vi "Set Data Channel Property - ALL.vi"(8 "error in":errorcluster, 10 "Item Informations array":T2[](array[typedef]), 11 "Item Ref in":T1 format="%.0x") -> (0 "error out":errorcluster)   [LabVIEW 2023, in "Vires VTD System Explorer.lvlib"]
uses:
  Vires VTD System Explorer.lvlib
  Item Informations.ctl
  <vilib>/NI VeriStand/Custom Device API/Custom Device Item Info.ctl
  <vilib>/NI VeriStand/Custom Device API/Custom Device Channel.ctl
  <vilib>/NI VeriStand/Custom Device API/Custom Device Channel Type.ctl
  Data Channel Custom Property.ctl
  <vilib>/NI VeriStand/Custom Device API/Custom Device Item Ref.ctl
  Shared/Constants.vi
  <vilib>/NI VeriStand/Custom Device API/Custom Device API.lvlib
  Shared/Vires VTD Shared.lvlib
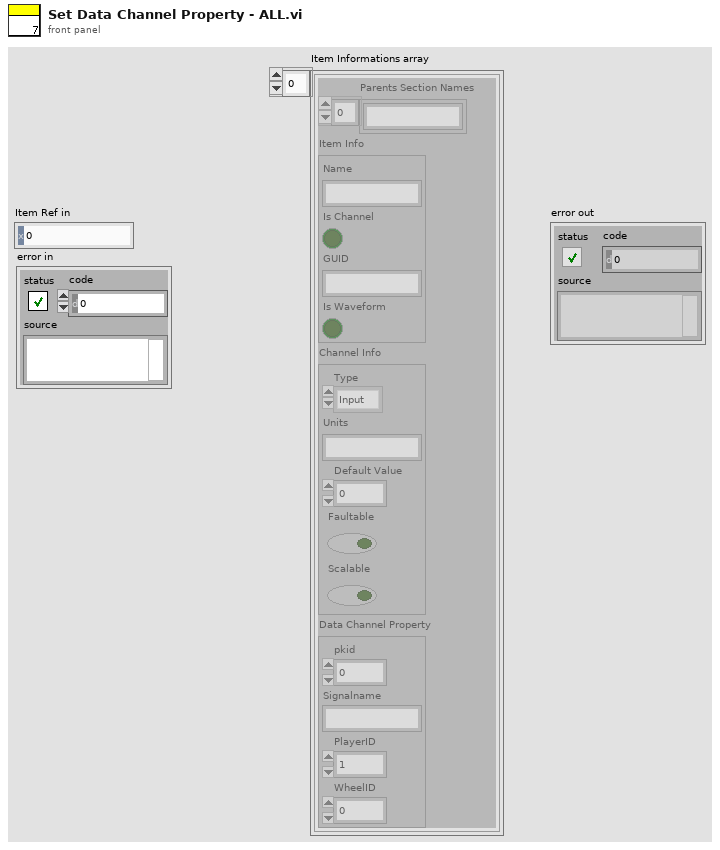
[diagram p1: front panel]
types:
  T1 = typedef "Custom Device API.lvlib/Custom Device Item Ref.ctl" = u64
  T2 = typedef "Vires VTD System Explorer.lvlib/Item Informations.ctl" = cluster{"Parents Section Names":string[], "Item Info":T3, "Channel Info":T4, "Data Channel Property":T6}
  T3 = typedef "Custom Device API.lvlib/Custom Device Item Info.ctl" = cluster{"Name":string, "Is Channel":bool, "GUID":string, "Is Waveform":bool}
  T4 = typedef "Custom Device API.lvlib/Custom Device Channel.ctl" = cluster{"Type":T5, "Units":string, "Default Value":dbl, "Faultable":bool, "Scalable":bool}
  T5 = typedef "Custom Device API.lvlib/Custom Device Channel Type.ctl" = enum16{"Input", "Output"}
  T6 = typedef "Vires VTD System Explorer.lvlib/Data Channel Custom Property.ctl" = cluster{"pkid":u32, "Signalname":string, "PlayerID":u8, "WheelID":i32}
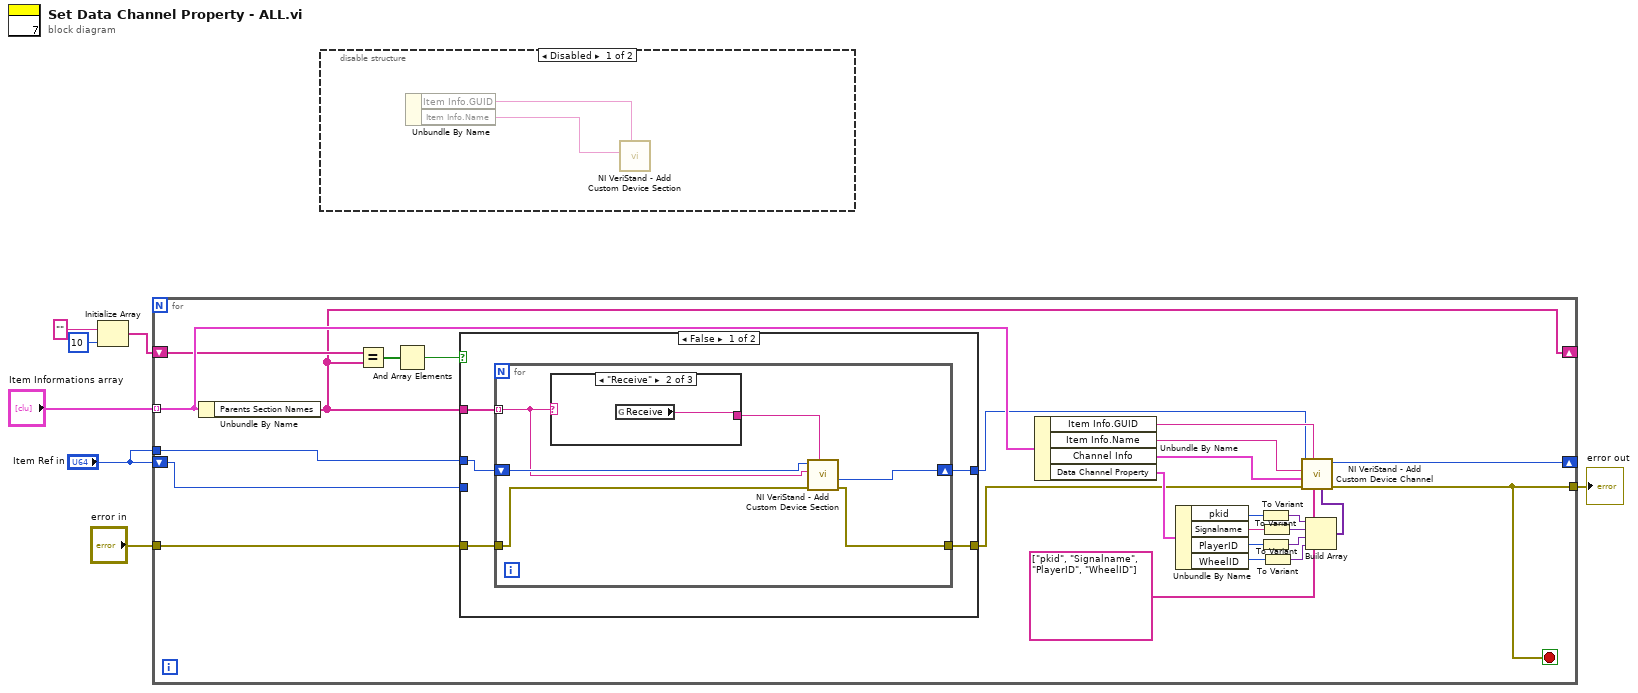
[diagram p0: block diagram]
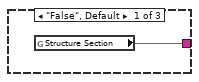
[diagram p3: hidden frame]
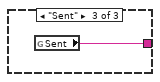
[diagram p4: hidden frame]
diagram:
  n1 = Initialize Array("" ("Parents Section Name"), 10 ("dimension size")) -> (w1:string[])
  n2 = for {
    tunnel: "Item Informations array" -> [w33] mode=indexing
    tunnel: [w32] -> w5
    tunnel: "error in" -> [w13]
    tunnel: "Item Ref in" -> [w14]
    shift-right: [w8] -> _
    shift-left: w1 -> [w17]
    shift-right: [w10] -> _
    shift-left: "Item Ref in" -> [w9]
    stop <- w32 stop-if-true
    n3 = Unbundle By Name(w33) -> ("Parents Section Names"=w8:string[])
    n4 = Equal?(x=w17, y=w8) -> (x = y?=w16:bool[])
    n5 = And Array Elements(Boolean array=w16) -> (logical AND=w15:bool)
    n6 = case shown="False" w15 {
      tunnel: w14 -> [w36 _]
      tunnel: w13 -> [w37 w49]
      tunnel: [w34 w49] -> w12
      tunnel: w8 -> [w38 _]
      tunnel: [w35 w48] -> w11
      tunnel: w9 -> [_ w48]
      frame False {
        n7 = for {
          tunnel: w38 -> [w39] mode=indexing
          tunnel: w37 -> [w41]
          shift-right: [w42] -> w35
          shift-left: w36 -> [w43]
          tunnel: [w40] -> w34
          n8 = case shown="\"Receive\"" w39 {
            tunnel: [w45 w46 w47] -> w44
            frame "False", Default {
              n9 = global read "Constants.vi" "Structure Section"() -> (w45:string)
            }
            frame "Receive" {
              n10 = global read "Constants.vi" "Receive"() -> (w46:string)
            }
            frame "Sent" {
              n11 = global read "Constants.vi" "Sent"() -> (w47:string)
            }
          }
          n12 = call <vilib>:"NI VeriStand - Add Custom Device Section.vi"("GUID (Default Section)"=w44, "error in (no error)"=w41, "Section Name"=w39, "Parent Ref in"=w43) -> ("error out"=w40:errorcluster, "Section Ptr"=w42:T1)  [unwired: 4 in, 2 out]
        }
      }
      frame True {
      }
    }
    n13 = Unbundle By Name(w33) -> ("Item Info.GUID"=w30:string, "Item Info.Name"=w31:string, "Channel Info"=w29:T4, "Data Channel Property"=w28:T6)
    n14 = Unbundle By Name(w28) -> ("pkid"=w22:u32, "Signalname"=w21:string, "PlayerID"=w20:u8, "WheelID"=w19:i32)
    n15 = To Variant(anything=w22) -> (Variant=w25:variant)
    n16 = To Variant(anything=w20) -> (Variant=w24:variant)
    n17 = To Variant(anything=w21) -> (Variant=w23:variant)
    n18 = To Variant(anything=w19) -> (Variant=w26:variant)
    n19 = Build Array(w25, w23, w24, w26) -> (w18:variant[])
    n20 = call <vilib>:"NI VeriStand - Add Custom Device Channel.vi"("Property Values"=w18, "Property names"=string[] ["pkid", "Signalname", "PlayerID", "WheelID"], "GUID (Default Channel)"=w30, "error in (no error)"=w12, "Channel"=w29, "Channel Name"=w31, "Parent Ref in"=w11) -> ("error out"=w32:errorcluster, "Parent Ref out"=w10:T1)  [unwired: 1 in, 2 out]
  }
  "error out" <- w5
  n21 = disable-structure shown="Disabled" {
    frame Disabled {
      n22 = Unbundle By Name() -> ("Item Info.GUID"=w50:string, "Item Info.Name"=w51:string)  [unwired: 1 in]
      n23 = call <vilib>:"NI VeriStand - Add Custom Device Section.vi"("GUID (Default Section)"=w50, "Section Name"=w51) -> ()  [unwired: 6 in, 4 out]
    }
    frame Enabled {
    }
  }
